vi "_Pull Controls Value to DPs(Refmgr).vi"(6 "sync DPs?(T)":bool=TRUE, 7 "VIRef(Caller VI)":refnum<k1>, 8 "error in (no error)":errorcluster, 9 "force update(F)":bool, 11 "SILAPI In":refnum<k1>) -> (0 "error out":errorcluster, 1 "Binded DPs":string[](array[string]), 3 "SILAPI Out":refnum<k1>)   [LabVIEW 2017, in "TagDB RefManager.lvlib"]
uses:
  TagDB RefManager.lvlib
  230c0da9-b6e4-44e0-8cb2-fe6bdec026ba.vi
  a90990ad-2366-4051-9646-140e847e3682.vi
  be640558-f0fc-44bb-96cd-108508b5fbdb.vi
  17cf8676-e257-4f33-957d-6af3ca117314.vi
  6c796322-1d76-4bdd-9aa2-7f47adde5471.vi
  024ec822-42c1-4cee-abf5-dbe2fbe4f70a.vi
  <userlib>/_NEVSTOP/TagDB/_Support/DataAccess/_NameCacher.vi
  <userlib>/_NEVSTOP/TagDB/_Support/Error/_[error50002]Invalid DataType.vi
  <userlib>/_NEVSTOP/TagDB/_Support/Error/_[error50000]Invalid DB REF.vi
  <userlib>/_NEVSTOP/TagDB/_Support/DataAccess/TagDB Ref to DVR.vi
  <userlib>/_NEVSTOP/TagDB/_Support/URL/TRIM-BOTH-SPACE.vi
  17cf8676-e257-4f33-957d-6af3ca117314.vi/1b47866c-8e2d-43a7-815f-8cf18635e5a1.vi
  6c796322-1d76-4bdd-9aa2-7f47adde5471.vi/1b47866c-8e2d-43a7-815f-8cf18635e5a1.vi
  <userlib>/_NEVSTOP/TagDB/_Support/DataAccess/data-Write.vi
  <userlib>/_NEVSTOP/TagDB/_Support/Change Detector/TagDB dbChanged.vi
  <userlib>/_NEVSTOP/TagDB/_Support/Error/_Clear Errors.vi
  17cf8676-e257-4f33-957d-6af3ca117314.vi/1b47866c-8e2d-43a7-815f-8cf18635e5a1.vi/29b2ea6d-6d7f-4e4a-ad31-a5cb760462c7.vi
  <userlib>/_NEVSTOP/TagDB/API/TagDB-Status.vi
  6c796322-1d76-4bdd-9aa2-7f47adde5471.vi/1b47866c-8e2d-43a7-815f-8cf18635e5a1.vi/29b2ea6d-6d7f-4e4a-ad31-a5cb760462c7.vi
  <userlib>/_NEVSTOP/TagDB/_Support/DataAccess/_datatypeChecker.vi
  <userlib>/_NEVSTOP/TagDB/_Support/Error/_Build Error Cluster.vi
  <vilib>/Utility/Data Type/Get Type Information.vi
  <userlib>/_NEVSTOP/TagDB/TagDB.lvlib
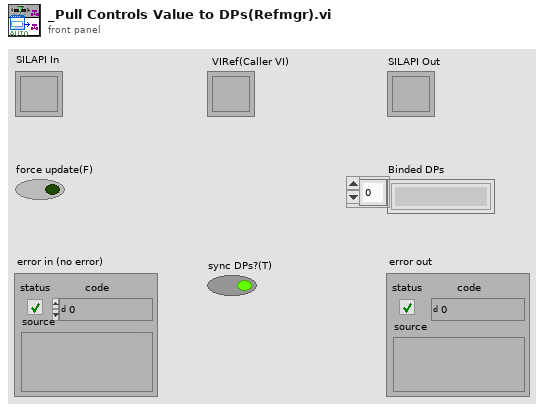
[diagram p1: front panel]
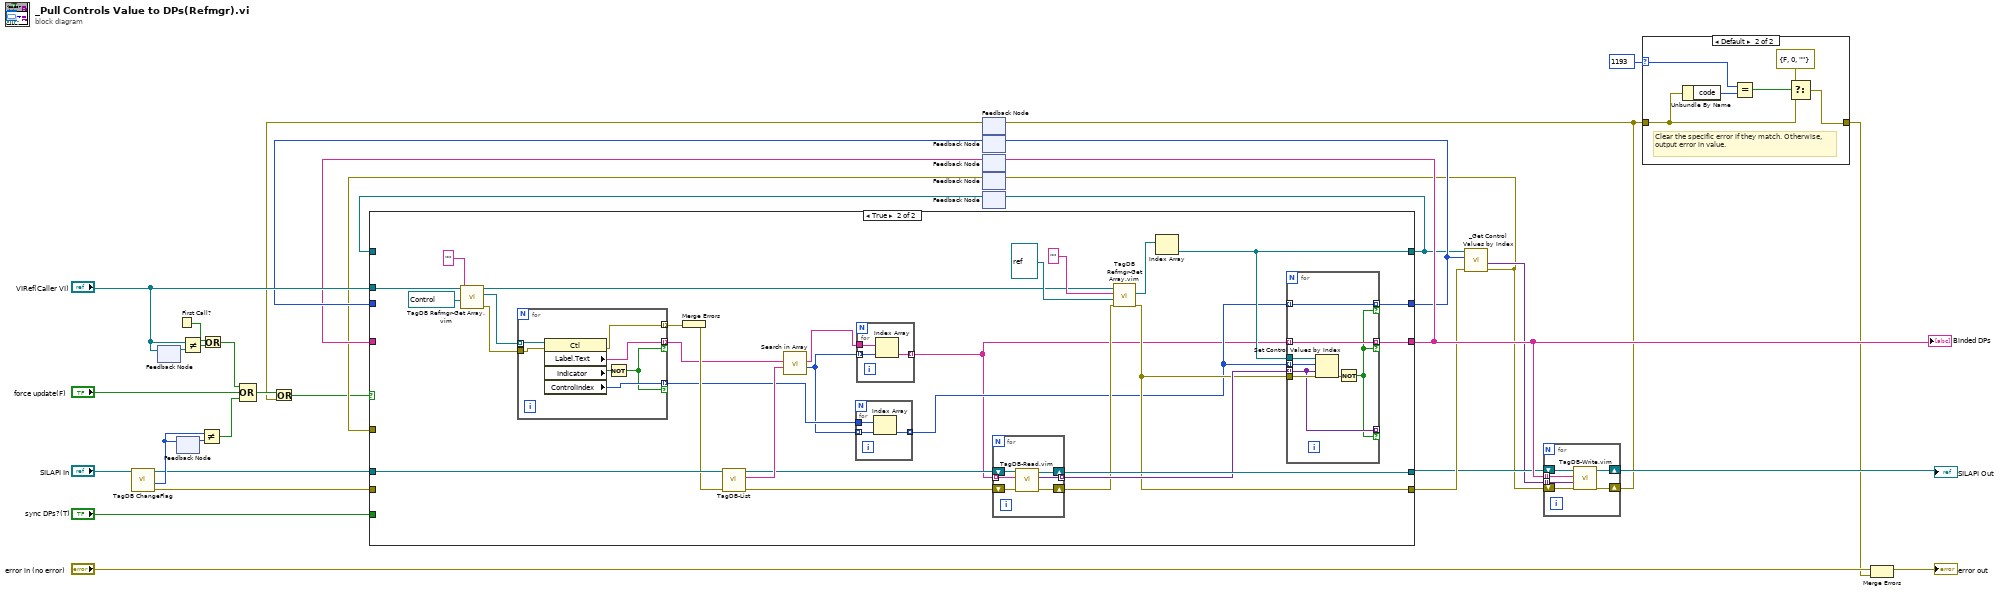
[diagram p0: block diagram]
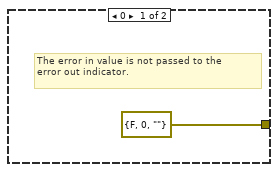
[diagram p2: hidden frame]
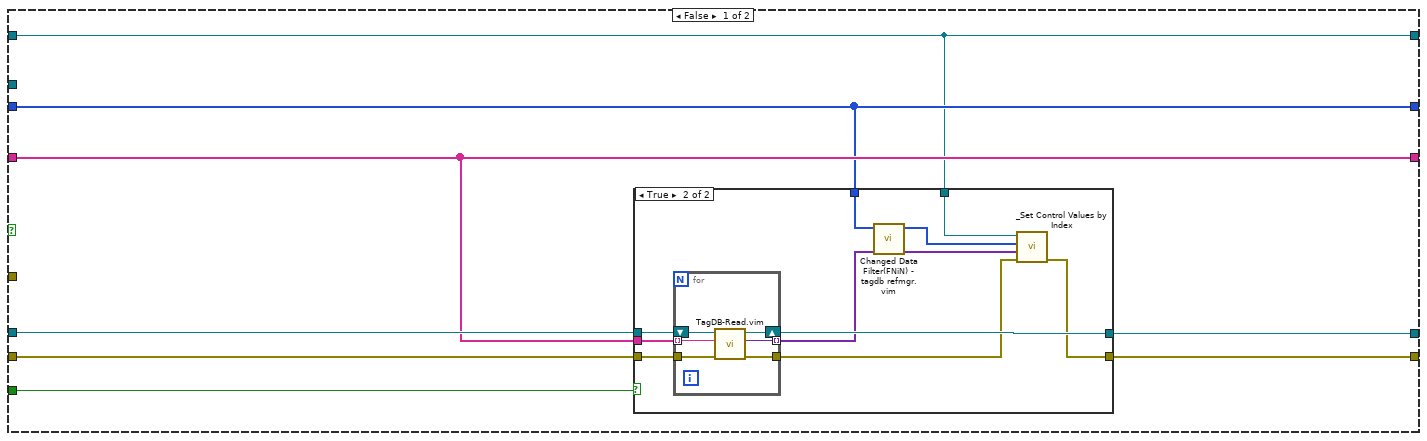
[diagram p3: hidden frame]
diagram:
  n1 = call <userlib>:"TagDB ChangeFlag.vi"("DB Ref"="SILAPI In") -> ("error in (no error) (dup)"=w4:errorcluster, "Item Change Timestamp"=w6:u64, "DB Ref (dup)"=w5:refnum<k1>)  [unwired: 7 in, 1 out]
  n2 = feedback #1() -> (w11:refnum<k1>)  [unwired: 1 in]
  n3 = feedback-in #1("VIRef(Caller VI)") -> ()
  n4 = First Call?() -> (First Call?: T/F=w9:bool)
  n5 = feedback #2() -> (w7:u64)  [unwired: 1 in]
  n6 = feedback-in #2(w6) -> ()
  n7 = Not Equal?(x="VIRef(Caller VI)", y=w11) -> (x != y?=w10:bool)
  n8 = Not Equal?(x=w6, y=w7) -> (x != y?=w3:bool)
  n9 = Or(x=w9, y=w10) -> (x .or. y?=w8:bool)
  n10 = Compound Arithmetic op=OR(w8, "force update(F)", w3) -> (w23:bool)
  n11 = feedback #3() -> (w18:errorcluster)  [unwired: 1 in]
  n12 = Or(x=w23, y=w18) -> (x .or. y?=w19:bool)
  n13 = feedback #4() -> (w24:i32[])  [unwired: 1 in]
  n14 = feedback #5() -> (w22:string[])  [unwired: 1 in]
  n15 = feedback #6() -> (w21:errorcluster)  [unwired: 1 in]
  n16 = feedback #7() -> (w12:refnum<vi>)  [unwired: 1 in]
  n17 = case shown="True" w19 {
    tunnel: [w35 w68] -> w13
    tunnel: "VIRef(Caller VI)" -> [_ w76]
    tunnel: [w37 w83] -> w25
    tunnel: w24 -> [w37 _]
    tunnel: [w40 w84] -> w27
    tunnel: w22 -> [w40 _]
    tunnel: w5 -> [w41 w88]
    tunnel: [w38 w69] -> w16
    tunnel: w21 -> [_ _]
    tunnel: [w39 w86] -> w15
    tunnel: "sync DPs?(T)" -> [w36 _]
    tunnel: w12 -> [w35 _]
    tunnel: w4 -> [w34 _]
    frame False {
      n18 = case shown="True" w36 {
        tunnel: w41 -> [w43 w54]
        tunnel: w40 -> [_ w53]
        tunnel: [w43 w52] -> w39
        tunnel: w35 -> [_ w51]
        tunnel: [w42 w49] -> w38
        tunnel: w37 -> [_ w46]
        tunnel: w34 -> [w42 w44]
        frame False {
        }
        frame True {
          n19 = for {
            tunnel: w53 -> [w59] mode=indexing
            tunnel: [w57] -> w50
            tunnel: [w56] -> w48 mode=indexing
            shift-right: [w58] -> w52
            shift-left: w54 -> [w60]
            tunnel: w44 -> [w55]
            n20 = call "TagDB-Read.vim"("error in (no error)"=w55, "name"=w59, "TagDB"=w60) -> ("error out"=w57:errorcluster, "Value"=w56:variant, "TagDB(dup)"=w58:refnum<k1>)  [unwired: 3 in, 3 out]
          }
          n21 = call "Changed Data Filter(FNiN) - tagdb refmgr.vim"("checked data"=w48, "1"=w46) -> ("data"=w47:variant[], "1 out"=w45:i32[])  [unwired: 6 in, 2 out]
          n22 = call <userlib>:"_Set Control Values by Index.vi"("error in (no error)"=w50, "data values"=w47, "control indexes"=w45, "VI Refnum"=w51) -> ("error out"=w49:errorcluster)  [unwired: 7 in]
        }
      }
    }
    frame True {
      n23 = call "TagDB Refmgr-Get Array.vim"("Type"=refnum<vi> refnum, "RegExp"="", "DB Ref"=w76) -> ("error out"=w75:errorcluster, "References"=w74:refnum<vi>[], "DB Ref(dup)"=w67:refnum<k1>)  [unwired: 5 in, 1 out]
      n24 = for {
        tunnel: w74 -> [w107] mode=indexing
        tunnel: [w106] -> w63 mode=indexing if=w101
        tunnel: [w105] -> w66 mode=indexing if=w101
        tunnel: [w103] -> w82 mode=indexing
        tunnel: w75 -> [w102]
        n25 = property class="Ctl"(reference=w107, error in=w102) -> (error out=w103:errorcluster, "Label.Text"=w106:string, "Indicator"=w104:bool, "ControlIndex"=w105:i32)  [unwired: 1 out]
        n26 = Not(x=w104) -> (.not. x?=w101:bool)
      }
      n27 = Merge Errors(w82) -> (w81:errorcluster)
      n28 = call <userlib>:"TagDB-List.vi"("error in (no error)"=w81, "TagDB"=w88) -> ("error out"=w87:errorcluster, "names"=w80:string[], "TagDB(dup)"=w79:refnum<k1>)  [unwired: 6 in, 1 out]
      n29 = call "Search in Array.vi"("items to filter"=w80, "array"=w63) -> ("item Indexs"=w64:i32[], "array(dup)"=w61:string[])  [unwired: 4 in]
      n30 = for {
        tunnel: w64 -> [w94] mode=indexing
        tunnel: w66 -> [w93]
        tunnel: [w92] -> w65 mode=indexing
        n31 = Index Array(array=w93, index=w94) -> (element=w92:i32)
      }
      n32 = for {
        tunnel: w64 -> [w91] mode=indexing
        tunnel: w61 -> [w90]
        tunnel: [w89] -> w62 mode=indexing
        n33 = Index Array(array=w90, index=w91) -> (element=w89:string)
      }
      n34 = for {
        tunnel: [w98] -> w85 mode=indexing
        tunnel: w62 -> [w96] mode=indexing
        shift-right: [w97] -> w70
        shift-left: w87 -> [w100]
        shift-right: [w99] -> w86
        shift-left: w79 -> [w95]
        n35 = call "TagDB-Read.vim"("error in (no error)"=w100, "name"=w96, "TagDB"=w95) -> ("error out"=w97:errorcluster, "Value"=w98:variant, "TagDB(dup)"=w99:refnum<k1>)  [unwired: 3 in, 3 out]
      }
      n36 = call "TagDB Refmgr-Get Array.vim"("error in (no error)"=w70, "Type"=refnum<vi> refnum ("Current VI Reference"), "RegExp"="", "DB Ref"=w67) -> ("error out"=w69:errorcluster, "References"=w71:refnum<vi>[])  [unwired: 4 in, 2 out]
      n37 = Index Array(array=w71) -> (element=w68:refnum<vi>)  [unwired: 1 in]
      n38 = for {
        tunnel: w68 -> [w115]
        tunnel: w65 -> [w114] mode=indexing
        tunnel: w85 -> [w110] mode=indexing
        tunnel: w69 -> [w113]
        tunnel: [w112] -> w84 mode=indexing if=w108
        tunnel: w62 -> [w112] mode=indexing
        tunnel: [w111] -> w83 mode=indexing if=w108
        tunnel: w65 -> [w111] mode=indexing
        tunnel: [w110] -> _ mode=indexing if=w108
        n39 = Set Control Values by Index(0:w115, 1:w114, 2:w110, 3:w113) -> (11:w109:errorcluster)
        n40 = Not(x=w109) -> (.not. x?=w108:bool)
      }
    }
  }
  "Binded DPs" <- w27
  n41 = feedback-in #4(w25) -> ()
  n42 = feedback-in #5(w27) -> ()
  n43 = feedback-in #7(w13) -> ()
  n44 = call <userlib>:"_Get Control Values by Index.vi"("error in (no error)"=w16, "control indexes"=w25, "VI Refnum"=w13) -> ("error out"=w1:errorcluster, "data values"=w2:variant[])  [unwired: 7 in]
  n45 = feedback-in #6(w1) -> ()
  n46 = for {
    shift-right: [w120] -> w28
    shift-left: w15 -> [w121]
    shift-right: [w116] -> w14
    shift-left: w1 -> [w119]
    tunnel: w27 -> [w118] mode=indexing
    tunnel: w2 -> [w117] mode=indexing
    n47 = call "TagDB-Write.vim"("error in (no error)"=w119, "Value"=w117, "tag"=w118, "TagDB"=w121) -> ("error out"=w116:errorcluster, "TagDB(dup)"=w120:refnum<k1>)  [unwired: 5 in, 1 out]
  }
  "SILAPI Out" <- w28
  n48 = feedback-in #3(w14) -> ()
  n49 = case shown="Default" 1193 ("specific error code to clear (0: all)") {
    selector: 1193 ("specific error code to clear (0: all)") -> [_ w127]
    tunnel: w14 -> [_ w126]
    tunnel: [errorcluster {"status"=FALSE, "code"=0, "source"=""} ("error constant") w123] -> w20
    frame 0 {
      # "The error in value is not passed to the\nerror out indicator."
    }
    frame Default {
      # "Clear the specific error if they match. Otherwise, output error in value."
      n50 = Unbundle By Name(w126) -> ("code"=w128:i32)
      n51 = Equal?(x=w127, y=w128) -> (x = y?=w124:bool)
      n52 = Select(t=errorcluster {"status"=FALSE, "code"=0, "source"=""} ("error constant"), s=w124, f=w126) -> (s? t:f=w123:errorcluster)
    }
  }
  n53 = Merge Errors("error in (no error)", w20) -> (→"error out":errorcluster)
